vi "PicoScope6000GetTimebase2.vi"(4 "Number of Samples":u32, 6 "Memory Segment":u32, 7 "Acquisition Settings":T1 {"postTriggerSamples" format="%_6p"; "preTriggerSamples" format="%_6p"}, 8 "error in (no error)":errorcluster, 11 "handle in":i16) -> (0 "error out":errorcluster, 3 "handle out":i16, 5 "Properties Panel":T2 {"Max Total Capture Time Available (sec)" format="%.3p"; "Sample Frequency" format="%.3p"; "Sample Internal" format="%.3p"; "Max Samples Available" format="%.3p"; "Total Capture Time (sec)" format="%.3p"})   [LabVIEW 2009]
uses:
  ps6000.dll
  shared/Acquisition Settings.ctl
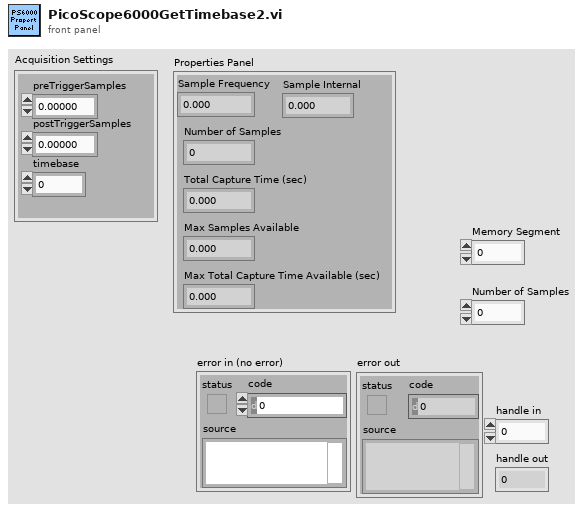
[diagram p1: front panel]
types:
  T1 = typedef "Acquisition Settings.ctl" = cluster{"preTriggerSamples":u64, "postTriggerSamples":u64, "timebase":u32}
  T2 = cluster{"Sample Frequency":sgl, "Sample Internal":sgl, "maxSamples":u32, "Number of Samples":u32, "Total Capture Time (sec) ":sgl, "Max Total Capture Time Available (sec)":sgl}
  T3 = cluster{sgl, sgl, "maxSamples":i32, "Number of Samples":u32, sgl, sgl}
  T4 = cluster{"status":bool, "code":u32, "source":string}
  T5 = cluster{sgl, sgl, "maxSamples":u32, "Number of Samples":u32, sgl, sgl}
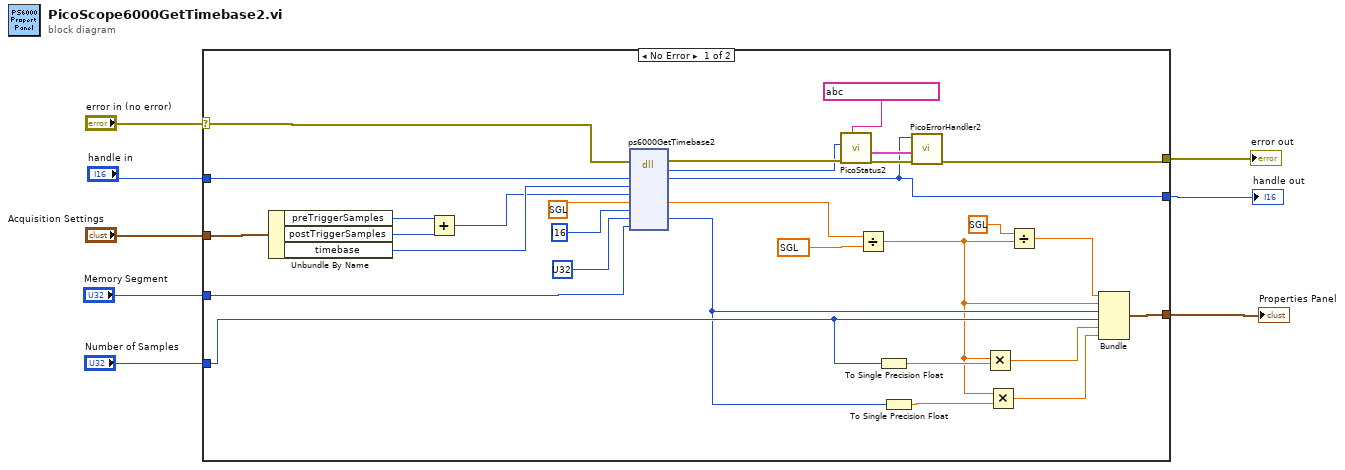
[diagram p0: block diagram]
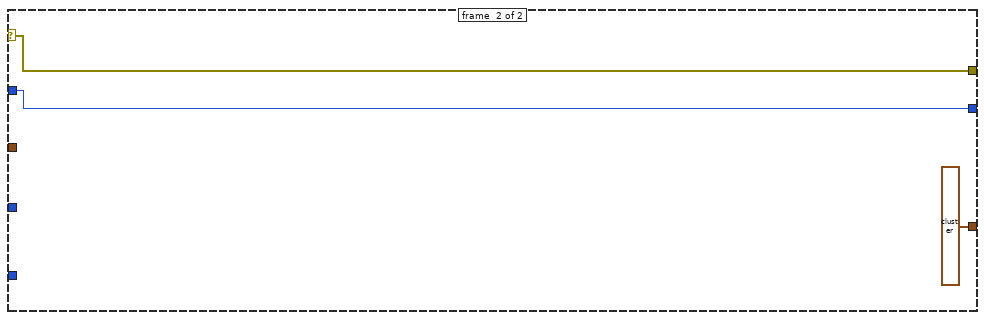
[diagram p2: hidden frame]
diagram:
  n1 = case shown="No Error" "error in (no error)" {
    selector: "error in (no error)" -> [w16 w41]
    tunnel: [w11 w41] -> w8
    tunnel: [w10 w40] -> w7
    tunnel: "Memory Segment" -> [w20 _]
    tunnel: "Number of Samples" -> [w29 _]
    tunnel: "handle in" -> [w33 w40]
    tunnel: "Acquisition Settings" -> [w32 _]
    tunnel: [w25 T3 ?] -> w2
    frame #0 {
      n2 = Unbundle By Name(w32) -> ("preTriggerSamples"=w34:u64, "postTriggerSamples"=w35:u64, "timebase"=w36:u32)
      n3 = Add(x=w34, y=w35) -> (x+y=w19:u64)
      n4 = dll-call lib="ps6000.dll" fn="ps6000GetTimebase2"(error in=w16, "handle"=w33, "timebase"=w36, "noSamples"=w19, "timeIntervalNanoseconds"=sgl ?, "oversample"=i16 ?, "maxSamples"=u32 ?, "segmentIndex"=w20) -> (error out=w13:errorcluster, "PICO_STATUS"=w9:u32, "handle"=w10:i16, "timeIntervalNanoseconds"=w37:sgl, "maxSamples"=w27:u32)  [unwired: 6 in, 1 out]
      n5 = call "PicoStatus2.vi"("PICO source"=string ? ("source"), "Error in"=w13, "PICO STATUS"=w9) -> ("error out"=w15:errorcluster, "PICO_STATUS out"=w14:T4)  [unwired: 5 in]
      n6 = Divide(x=w37, y=sgl ?) -> (x/y=w22:sgl)
      n7 = To Single Precision Float(number=w29) -> (single precision float=w31:sgl)
      n8 = To Single Precision Float(number=w27) -> (single precision float=w28:sgl)
      n9 = call "PicoErrorHandler2.vi"("error in (no error)"=w15, "PICO_STATUS in"=w14, "handle In"=w10) -> ("error out"=w11:errorcluster)  [unwired: 8 in]
      n10 = Multiply(x=w22, y=w31) -> (x*y=w30:sgl)
      n11 = Multiply(x=w22, y=w28) -> (x*y=w26:sgl)
      n12 = Divide(x=sgl ?, y=w22) -> (x/y=w23:sgl)
      n13 = Bundle(w23, w22, "maxSamples"=w27, "Number of Samples"=w29, w30, w26) -> (w25:T5)  [unwired: 1 in]
    }
    frame #1 {
    }
  }
  "error out" <- w8
  "handle out" <- w7
  "Properties Panel" <- w2
